vi "Sys_DAQ_Global.vi"() -> ()   [LabVIEW 2025, in "Keithley-DAQ6510 System Explorer.lvlib"]
uses:
  Keithley-DAQ6510 System Explorer.lvlib
panel:
  in  "Channel_list":string="Keithley-DAQ6510"
  in  "Keithley-DAQ6510":string="Keithley-DAQ6510"
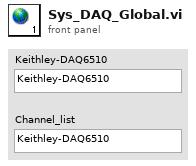
[diagram p1: front panel]
diagram:
